vi "Riccati_Input_Check.vi"(8 "R":T1, 9 "Q":T1, 10 "B":T1, 11 "A":T1) -> (0 "error out":errorcluster, 3 "Error":bool)   [LabVIEW 2019, in "Trajectory_Library.lvlib"]
doc: "This is an internal function, called only by the DARE routines.\n\nThis routine checks the inputs for validity prior to calling DARE.\n\nInputs\n - A -- A matrix\n - B -- B matrix\n - Q -- Q matrix\n - R -- R matrix\n\nOutput:\n - Error -- If TRUE, the input checks failed or in internal error occured.\n - Error out -- Error cluster"
uses:
  Trajectory_Library.lvlib
  <vilib>/Analysis/Matrix/Datatypes/RealMatrix.ctl
  <vilib>/Analysis/7linalg.llb/Eigenvalue and Vectors Output Option.ctl
  <vilib>/Analysis/7linalg.llb/Real Cholesky Factorization.vi
  <vilib>/Analysis/7linalg.llb/Real Transpose Matrix.vi
  <vilib>/Analysis/baseanly.llb/Full Cholesky Factorization.vi
  <vilib>/Analysis/baseanly.llb/Full Real Matrix Cholesky Factorization.vi
  <vilib>/Analysis/Matrix/Numeric/Subtract/Subtract - RM,RM.vi
  <vilib>/Analysis/Matrix/Numeric/Absolute Value/Absolute Value - RM.vi
  <vilib>/Analysis/7linalg.llb/Real Eigenvalues and Vectors.vi
  <vilib>/Analysis/NI_AALPro.lvlib
  <vilib>/Analysis/Matrix/NI_Matrix.lvlib
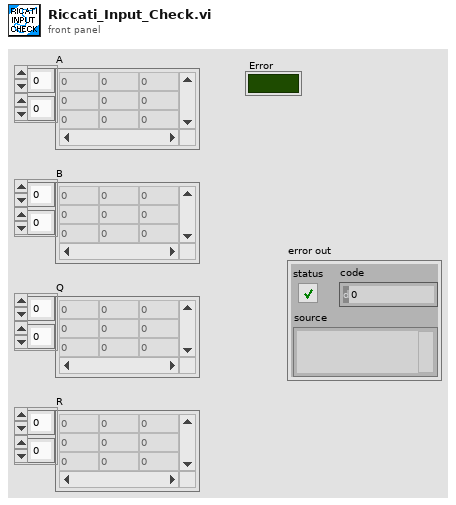
[diagram p1: front panel]
types:
  T1 = typedef "NI_Matrix.lvlib/RealMatrix.ctl" = dbl[][]
  T2 = typedef "NI_AALPro.lvlib/Eigenvalue and Vectors Output Option.ctl" = i32
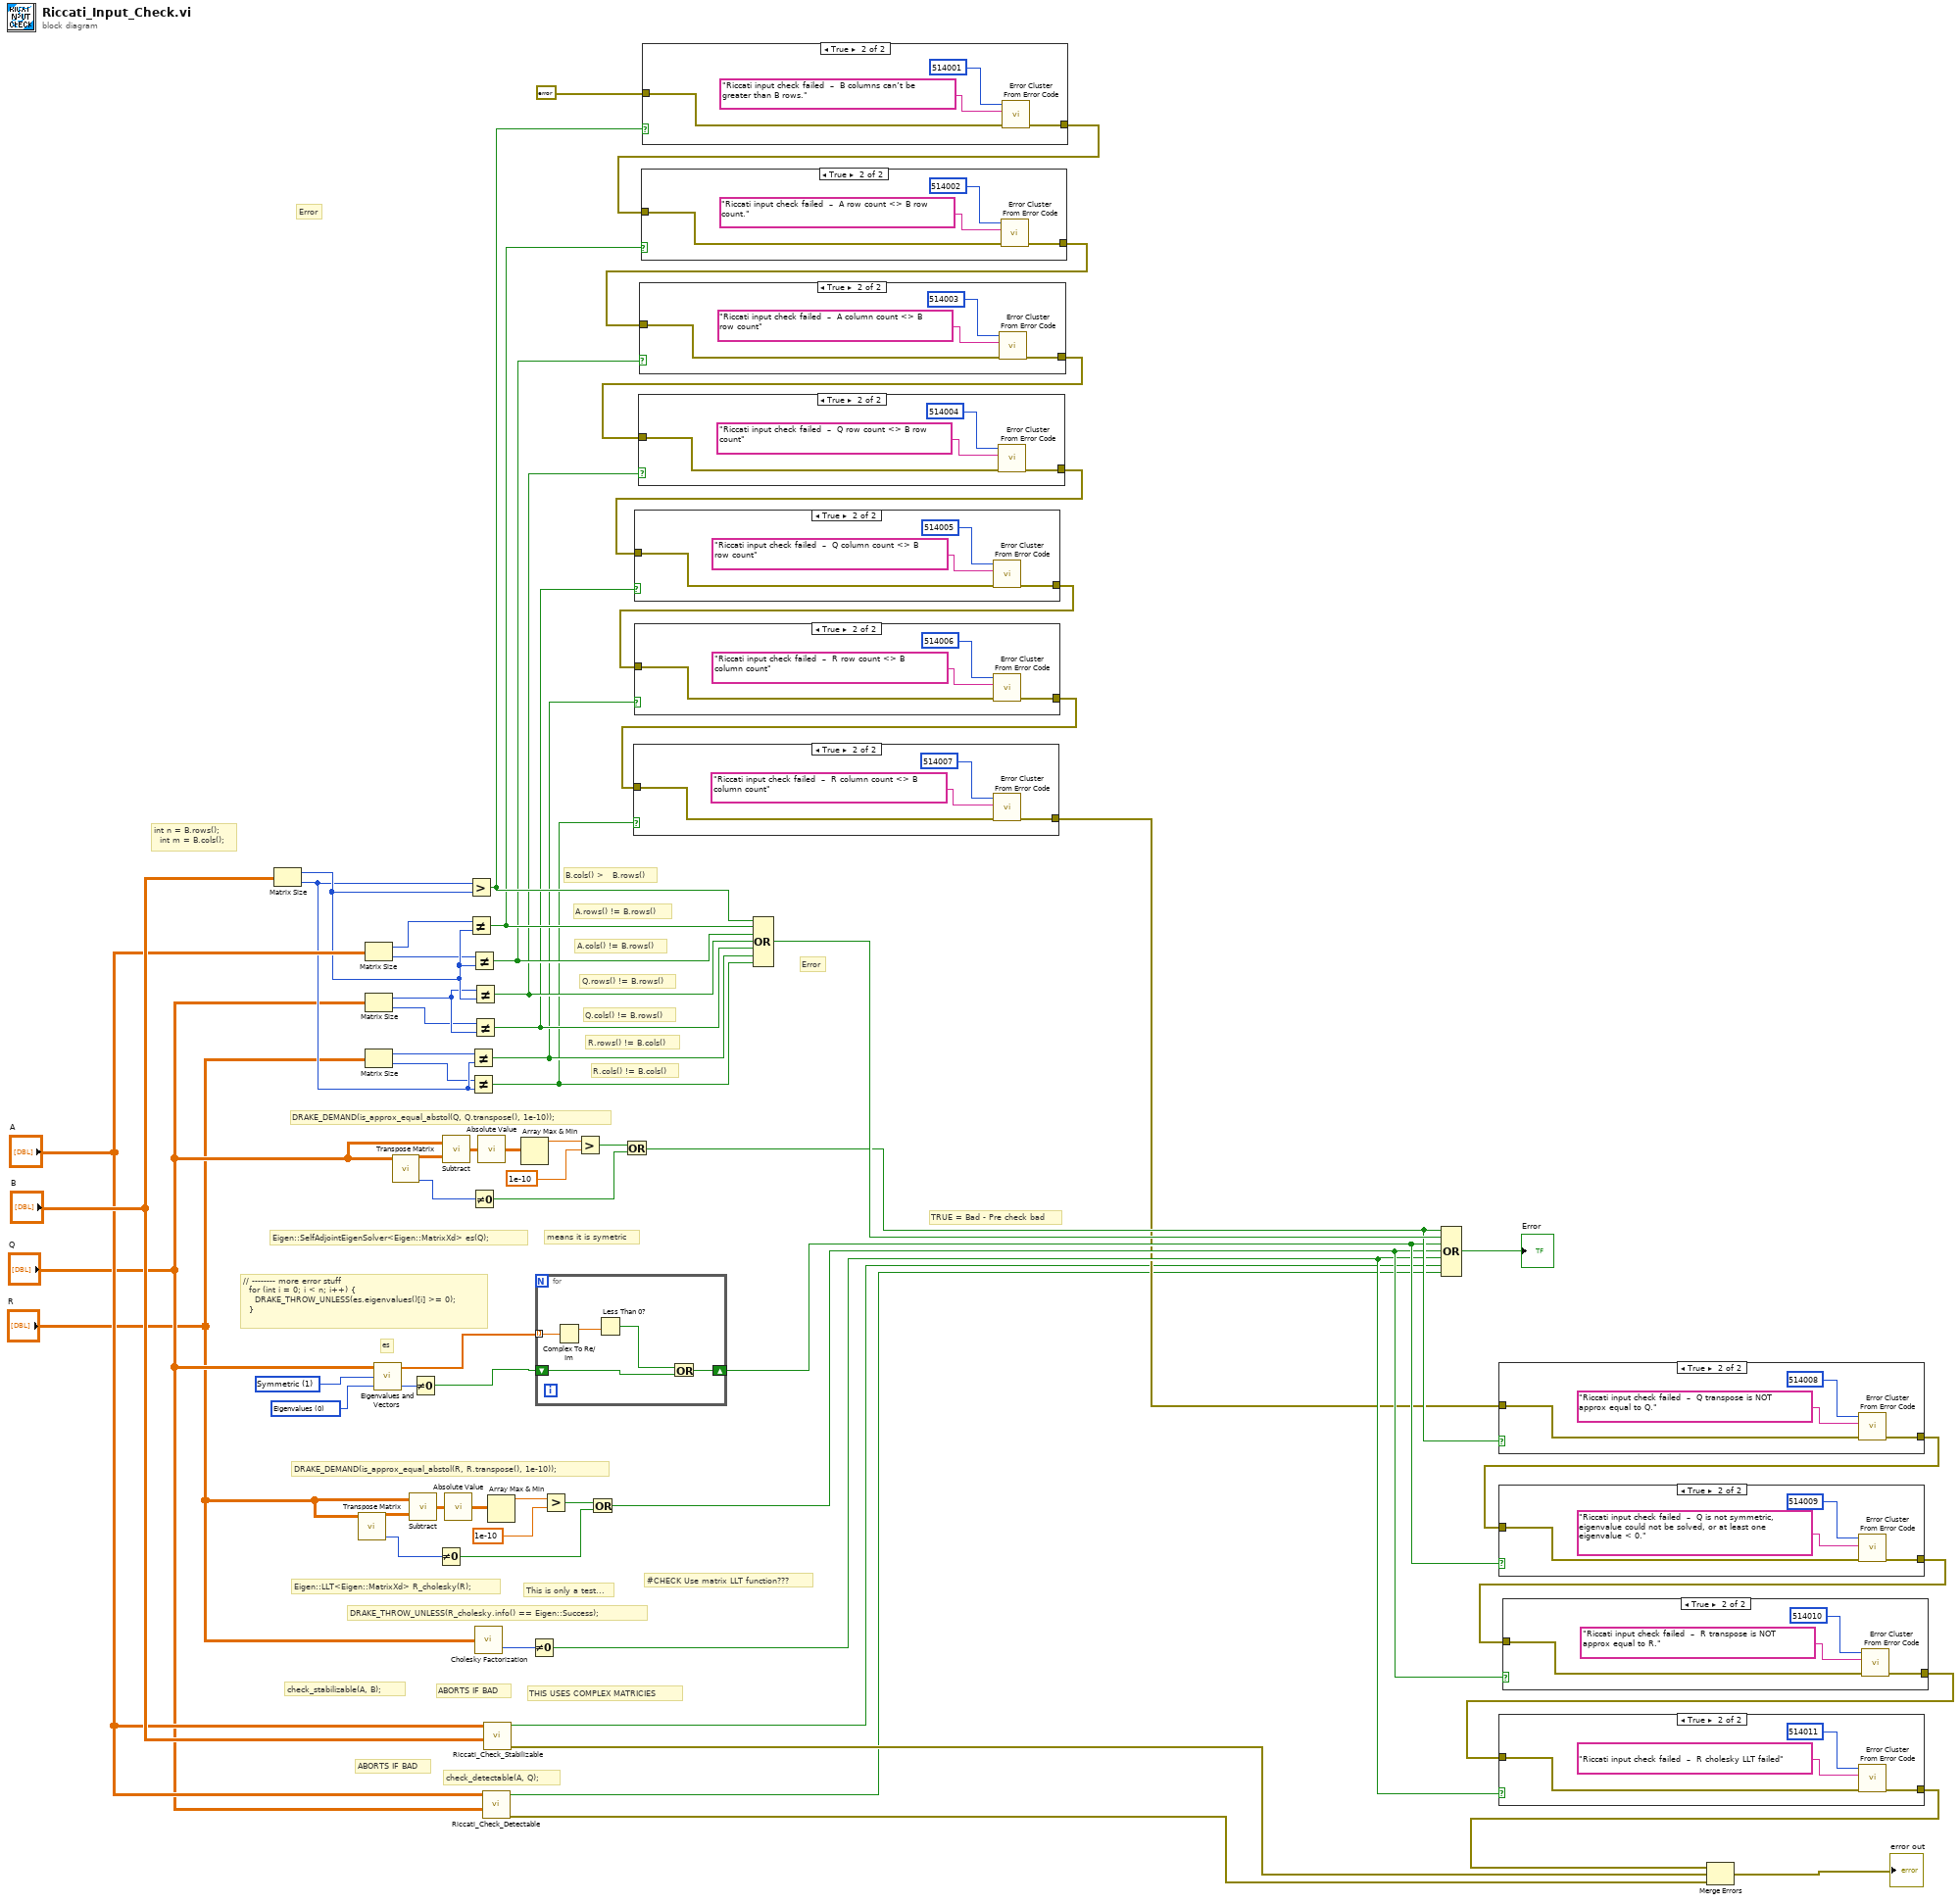
[diagram p0: block diagram]
diagram:
  w52 = 1 items=["General", "Symmetric"] ("matrix type")
  w51 = T2 0 items=["Eigenvalues", "Eigenvalues & Vectors"] ("output option")
  # "#CHECK Use matrix LLT function???"
  # "Error"
  # "DRAKE_DEMAND(is_approx_equal_abstol(R, R.transpose(), 1e-10));"
  # "R.cols() != B.cols()"
  # "R.rows() != B.cols()"
  # "Q.cols() != B.rows()"
  # "Q.rows() != B.rows()"
  # "A.cols() != B.rows()"
  # "A.rows() != B.rows()"
  # "B.cols() >   B.rows()"
  # "Error"
  # "TRUE = Bad - Pre check bad"
  # "DRAKE_DEMAND(is_approx_equal_abstol(Q, Q.transpose(), 1e-10));"
  # "int n = B.rows(); \n  int m = B.cols();"
  # "This is only a test..."
  # "ABORTS IF BAD"
  # "ABORTS IF BAD"
  # "check_stabilizable(A, B);"
  # "THIS USES COMPLEX MATRICIES"
  # "DRAKE_THROW_UNLESS(R_cholesky.info() == Eigen::Success);"
  # "// -------- more error stuff\n  for (int i = 0; i < n; i++) {\n    DRAKE_THROW_UNLESS(es.eigenvalues()[i] >= 0);\n  }"
  # "check_detectable(A, Q);"
  # "Eigen::LLT<Eigen::MatrixXd> R_cholesky(R);"
  # "es"
  # "means it is symetric"
  # "Eigen::SelfAdjointEigenSolver<Eigen::MatrixXd> es(Q);"
  n1 = Matrix Size(0:"B") -> (1:w60:i32, 2:w59:i32)
  n2 = call-poly <vilib>:"Transpose Matrix.vi"("Input Matrix"="R") -> ("error"=w37:i32, "Matrix Transpose"=w38:T1)  [unwired: 9 in]
  n3 = Matrix Size(0:"A") -> (1:w53:i32, 2:w54:i32)
  n4 = Matrix Size(0:"Q") -> (1:w56:i32, 2:w55:i32)
  n5 = Matrix Size(0:"R") -> (1:w57:i32, 2:w58:i32)
  n6 = call-poly <vilib>:"Eigenvalues and Vectors.vi"("output option"=w51, "matrix type"=w52, "Input Matrix"="Q") -> ("error"=w62:i32, "Eigenvalues"=w29:cdb[])  [unwired: 1 out]
  n7 = call-poly <vilib>:"Transpose Matrix.vi"("Input Matrix"="Q") -> ("error"=w45:i32, "Matrix Transpose"=w46:T1)  [unwired: 9 in]
  n8 = call-poly <vilib>:"Subtract.vi"("Real Matrix B"=w38, "Real Matrix A"="R") -> ("A - B"=w36:T1)
  n9 = Not Equal To 0?(x=w62) -> (x != 0?=w28:bool)
  n10 = Not Equal To 0?(x=w37) -> (x != 0?=w31:bool)
  n11 = call-poly <vilib>:"Subtract.vi"("Real Matrix B"=w46, "Real Matrix A"="Q") -> ("A - B"=w44:T1)
  n12 = call-poly <vilib>:"Absolute Value.vi"("Real Matrix A"=w36) -> ("|A|"=w35:T1)
  n13 = Greater?(x=w59, y=w60) -> (0:w48:bool)
  n14 = Not Equal?(x=w53, y=w60) -> (x != y?=w26:bool)
  n15 = Not Equal?(x=w57, y=w59) -> (x != y?=w17:bool)
  n16 = Not Equal?(x=w58, y=w59) -> (x != y?=w15:bool)
  n17 = Not Equal?(x=w54, y=w60) -> (x != y?=w25:bool)
  n18 = Not Equal To 0?(x=w45) -> (x != 0?=w39:bool)
  n19 = Not Equal?(x=w56, y=w60) -> (x != y?=w24:bool)
  n20 = Not Equal?(x=w55, y=w56) -> (x != y?=w19:bool)
  n21 = call-poly <vilib>:"Cholesky Factorization.vi"("A"="R") -> ("error"=w61:i32)  [unwired: 1 out]
  n22 = call-poly <vilib>:"Absolute Value.vi"("Real Matrix A"=w44) -> ("|A|"=w43:T1)
  n23 = call "Riccati_Check_Detectable.vi"("Q"="Q", "A"="A") -> ("error out"=w1:errorcluster, "Bad"=w3:bool)  [unwired: 3 in, 5 out]
  n24 = call "Riccati_Check_Stabilizable.vi"("B"="B", "A"="A") -> ("Error"=w4:errorcluster, "Bad"=w6:bool)  [unwired: 8 in]
  n25 = Array Max & Min(array=w35) -> (max value=w34:dbl)  [unwired: 3 out]
  n26 = Array Max & Min(array=w43) -> (max value=w42:dbl)  [unwired: 3 out]
  n27 = Not Equal To 0?(x=w61) -> (x != 0?=w11:bool)
  n28 = for {
    tunnel: w29 -> [w69] mode=indexing
    shift-right: [w67] -> w13
    shift-left: w28 -> [w66]
    n29 = Complex To Re/Im(x + iy=w69) -> (x=w68:dbl)  [unwired: 1 out]
    n30 = Less Than 0?(x=w68) -> (x < 0?=w65:bool)
    n31 = Or(x=w65, y=w66) -> (x .or. y?=w67:bool)
  }
  n32 = Greater?(x=w34, y=1e-10) -> (0:w32:bool)
  n33 = Greater?(x=w42, y=1e-10) -> (0:w40:bool)
  n34 = Or(x=w32, y=w31) -> (x .or. y?=w12:bool)
  n35 = Or(x=w40, y=w39) -> (x .or. y?=w14:bool)
  n36 = case shown="True" w48 {
    tunnel: errorcluster {"status"=FALSE, "code"=0, "source"=""} ("error constant") -> [w70 w72]
    tunnel: [w70 w71] -> w23
    frame False {
    }
    frame True {
      n37 = call <vilib>:"Error Cluster From Error Code.vi"("error in (no error)"=w72, "error message (\"\")"="Riccati input check failed  –  B columns can’t be greater than B rows." ("error message (\"\")"), "error code (0)"=514001) -> ("error out"=w71:errorcluster)  [unwired: 6 in]
    }
  }
  n38 = case shown="True" w26 {
    tunnel: w23 -> [w75 w77]
    tunnel: [w75 w76] -> w22
    frame False {
    }
    frame True {
      n39 = call <vilib>:"Error Cluster From Error Code.vi"("error in (no error)"=w77, "error message (\"\")"="Riccati input check failed  –  A row count <> B row count." ("error message (\"\")"), "error code (0)"=514002) -> ("error out"=w76:errorcluster)  [unwired: 6 in]
    }
  }
  n40 = case shown="True" w25 {
    tunnel: w22 -> [w80 w82]
    tunnel: [w80 w81] -> w21
    frame False {
    }
    frame True {
      n41 = call <vilib>:"Error Cluster From Error Code.vi"("error in (no error)"=w82, "error message (\"\")"="Riccati input check failed  –  A column count <> B row count" ("error message (\"\")"), "error code (0)"=514003) -> ("error out"=w81:errorcluster)  [unwired: 6 in]
    }
  }
  n42 = case shown="True" w24 {
    tunnel: w21 -> [w85 w87]
    tunnel: [w85 w86] -> w20
    frame False {
    }
    frame True {
      n43 = call <vilib>:"Error Cluster From Error Code.vi"("error in (no error)"=w87, "error message (\"\")"="Riccati input check failed  –  Q row count <> B row count" ("error message (\"\")"), "error code (0)"=514004) -> ("error out"=w86:errorcluster)  [unwired: 6 in]
    }
  }
  n44 = case shown="True" w19 {
    tunnel: w20 -> [w90 w92]
    tunnel: [w90 w91] -> w18
    frame False {
    }
    frame True {
      n45 = call <vilib>:"Error Cluster From Error Code.vi"("error in (no error)"=w92, "error message (\"\")"="Riccati input check failed  –  Q column count <> B row count" ("error message (\"\")"), "error code (0)"=514005) -> ("error out"=w91:errorcluster)  [unwired: 6 in]
    }
  }
  n46 = case shown="True" w17 {
    tunnel: w18 -> [w95 w97]
    tunnel: [w95 w96] -> w16
    frame False {
    }
    frame True {
      n47 = call <vilib>:"Error Cluster From Error Code.vi"("error in (no error)"=w97, "error message (\"\")"="Riccati input check failed  –  R row count <> B column count" ("error message (\"\")"), "error code (0)"=514006) -> ("error out"=w96:errorcluster)  [unwired: 6 in]
    }
  }
  n48 = case shown="True" w15 {
    tunnel: w16 -> [w100 w102]
    tunnel: [w100 w101] -> w10
    frame False {
    }
    frame True {
      n49 = call <vilib>:"Error Cluster From Error Code.vi"("error in (no error)"=w102, "error message (\"\")"="Riccati input check failed  –  R column count <> B column count" ("error message (\"\")"), "error code (0)"=514007) -> ("error out"=w101:errorcluster)  [unwired: 6 in]
    }
  }
  n50 = Compound Arithmetic op=OR(w48, w26, w25, w24, w19, w17, w15) -> (w49:bool)
  n51 = Compound Arithmetic op=OR(w14, w49, w13, w12, w11, w6, w3) -> (→"Error":bool)
  n52 = case shown="True" w14 {
    tunnel: w10 -> [w105 w107]
    tunnel: [w105 w106] -> w9
    frame False {
    }
    frame True {
      n53 = call <vilib>:"Error Cluster From Error Code.vi"("error in (no error)"=w107, "error message (\"\")"="Riccati input check failed  –  Q transpose is NOT approx equal to Q." ("error message (\"\")"), "error code (0)"=514008) -> ("error out"=w106:errorcluster)  [unwired: 6 in]
    }
  }
  n54 = case shown="True" w13 {
    tunnel: w9 -> [w110 w112]
    tunnel: [w110 w111] -> w8
    frame False {
    }
    frame True {
      n55 = call <vilib>:"Error Cluster From Error Code.vi"("error in (no error)"=w112, "error message (\"\")"="Riccati input check failed  –  Q is not symmetric, eigenvalue could not be solved, or at least one eigenvalue < 0." ("error message (\"\")"), "error code (0)"=514009) -> ("error out"=w111:errorcluster)  [unwired: 6 in]
    }
  }
  n56 = case shown="True" w12 {
    tunnel: w8 -> [w115 w117]
    tunnel: [w115 w116] -> w7
    frame False {
    }
    frame True {
      n57 = call <vilib>:"Error Cluster From Error Code.vi"("error in (no error)"=w117, "error message (\"\")"="Riccati input check failed  –  R transpose is NOT approx equal to R." ("error message (\"\")"), "error code (0)"=514010) -> ("error out"=w116:errorcluster)  [unwired: 6 in]
    }
  }
  n58 = case shown="True" w11 {
    tunnel: w7 -> [w120 w122]
    tunnel: [w120 w121] -> w5
    frame False {
    }
    frame True {
      n59 = call <vilib>:"Error Cluster From Error Code.vi"("error in (no error)"=w122, "error message (\"\")"="Riccati input check failed  –  R cholesky LLT failed" ("error message (\"\")"), "error code (0)"=514011) -> ("error out"=w121:errorcluster)  [unwired: 6 in]
    }
  }
  n60 = Merge Errors(w5, w4, w1) -> (→"error out":errorcluster)
